vi "WaitOnListener.vi"(8 "error in (no error)":errorcluster, 10 "timeout ms":i32=500, 11 "TCPIP in":refnum<class "TCPIP.lvclass">) -> (0 "error out":errorcluster, 3 "TCPIP out":refnum<class "TCPIP.lvclass">)   [LabVIEW 2018, in "TCPIP.lvclass"]
uses:
  TCPIP.lvclass
  TCPIP.lvclass/TCPIP.ctl
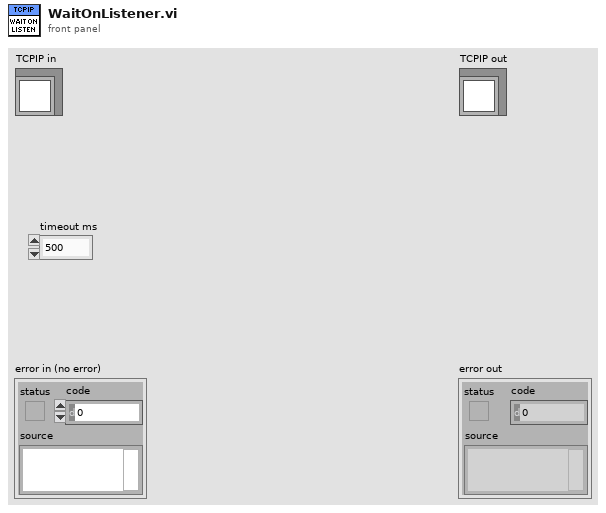
[diagram p1: front panel]
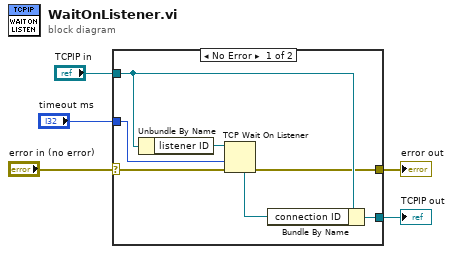
[diagram p0: block diagram]
diagram:
  n1 = case shown="No Error" "error in (no error)" {
    selector: "error in (no error)" -> [w9 w14]
    tunnel: [w8 w14] -> w4
    tunnel: [w12 w13] -> w2
    tunnel: "TCPIP in" -> [w11 w13]
    tunnel: "timeout ms" -> [w7 _]
    frame No Error {
      n2 = Unbundle By Name(w11) -> ("listener ID"=w10:refnum<k5>)
      n3 = TCP Wait On Listener(8:w9, 9:w7, 11:w10) -> (0:w8:errorcluster, 4:w6:refnum<k5>)  [unwired: 1 in, 3 out]
      n4 = Bundle By Name(cluster=w11, "connection ID"=w6) -> (w12:refnum<class "TCPIP.lvclass">)
    }
    frame Error {
    }
  }
  "error out" <- w4
  "TCPIP out" <- w2
